vi "Build_Asylum_SetSTFC.vi"(6 "trigger":cluster{"Value":dbl, "greaterOrLesser":dbl}, 7 "eventString":string, 8 "error in (no error)":errorcluster, 9 "inChannelString":string, 10 "time":dbl, 11 "z":cluster{"Start":dbl, "End":dbl}) -> (0 "error out":errorcluster, 3 "Command":string)   [LabVIEW 2019]
panel:
  in  "callback":string
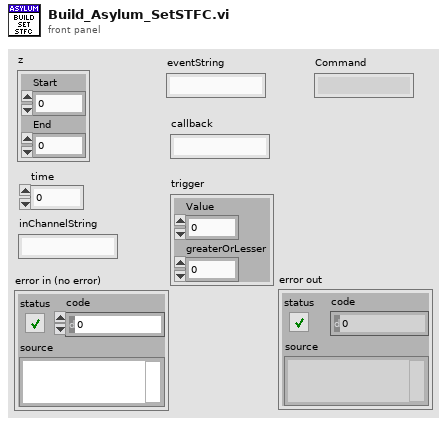
[diagram p1: front panel]
types:
  T1 = cluster{"Value":string, "greaterOrLesser":string}
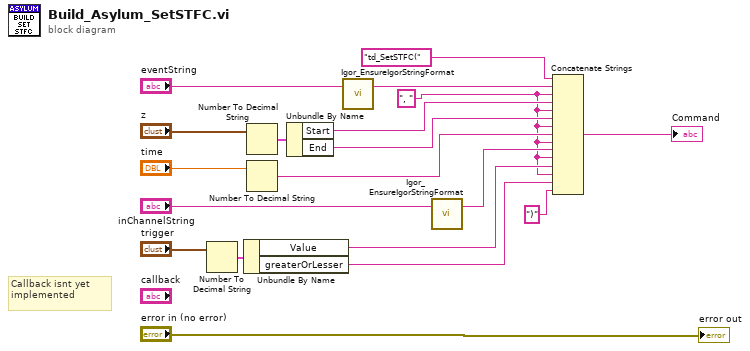
[diagram p0: block diagram]
diagram:
  w4 = ", " ("string")
  # "Callback isnt yet implemented"
  n1 = Number To Decimal String(number="trigger") -> (decimal integer string=w13:T1)  [unwired: 1 in]
  n2 = Unbundle By Name(w13) -> ("Value"=w6:string, "greaterOrLesser"=w5:string)
  n3 = Number To Decimal String(number="z") -> (decimal integer string=w14:cluster{"Start":string, "End":string})  [unwired: 1 in]
  n4 = Number To Decimal String(number="time") -> (decimal integer string=w8:string)  [unwired: 1 in]
  n5 = Unbundle By Name(w14) -> ("Start"=w10:string, "End"=w9:string)
  n6 = call <userlib>:"Igor_EnsureIgorStringFormat.vi"("Value"="eventString") -> ("Value"=w17:string)  [unwired: 2 in]
  n7 = call <userlib>:"Igor_EnsureIgorStringFormat.vi"("Value"="inChannelString") -> ("Value"=w7:string)  [unwired: 2 in]
  n8 = Concatenate Strings("td_SetSTFC(" ("string"), w17, w4, w10, w4, w9, w4, w8, w4, w7, w4, w6, w4, w5, ")" ("string")) -> (→"Command":string)
  "error out" <- "error in (no error)"
